vi "DAQ Stop.vi"(8 "Error In":errorcluster caption="错误输入", 10 "Sample Settings":T1={"设备信息"={"初始索引子集"=[], "模拟信号采集通道"="Dev1", "光控设备"="", "数字-光控"="", "数字-供电"="", "光电设备分离？"=FALSE, "光谱保存路径"=path "", "7环?"=FALSE}, "测量控制"={"测头拿起"=FALSE, "是否保存"=FALSE, "测头供电"=TRUE, "测头出光"=TRUE}, "测量"={"每波长测量次数"=5, "波长"=[1050, 1213, 1314, 1409, 1550, 1609], "起始周期"=0, "起始测量周期"=0}, "等待"={"等待时间(s)"=0.0, "等待方式"=FALSE, "每x周期/点等待"=8, "等待时"=enum."无电无光"}, "校准"={"暗电流校准值初值"=[], "温度校准值"=[0.0, 0.0, 0.0, 0.0, 0.0, 0.0, 0.00013, 0.00013, 0.00013, 0.00013, 0.00013, 0.00013]}, "图表相关"={"文件-时间"=""}}) -> (0 "Error Out":errorcluster caption="错误输出")   [LabVIEW 2017, in "UI-无创.lvlib" / "Acquisition.lvlib"]
uses:
  Acquisition.lvlib
  Supports/Sample Settings.ctl
  <vilib>/DAQmx/write.llb/DAQmx Write (Digital U32 1Chan 1Samp).vi
  <vilib>/DAQmx/miscellaneous.llb/DAQmx Fill In Error Info.vi
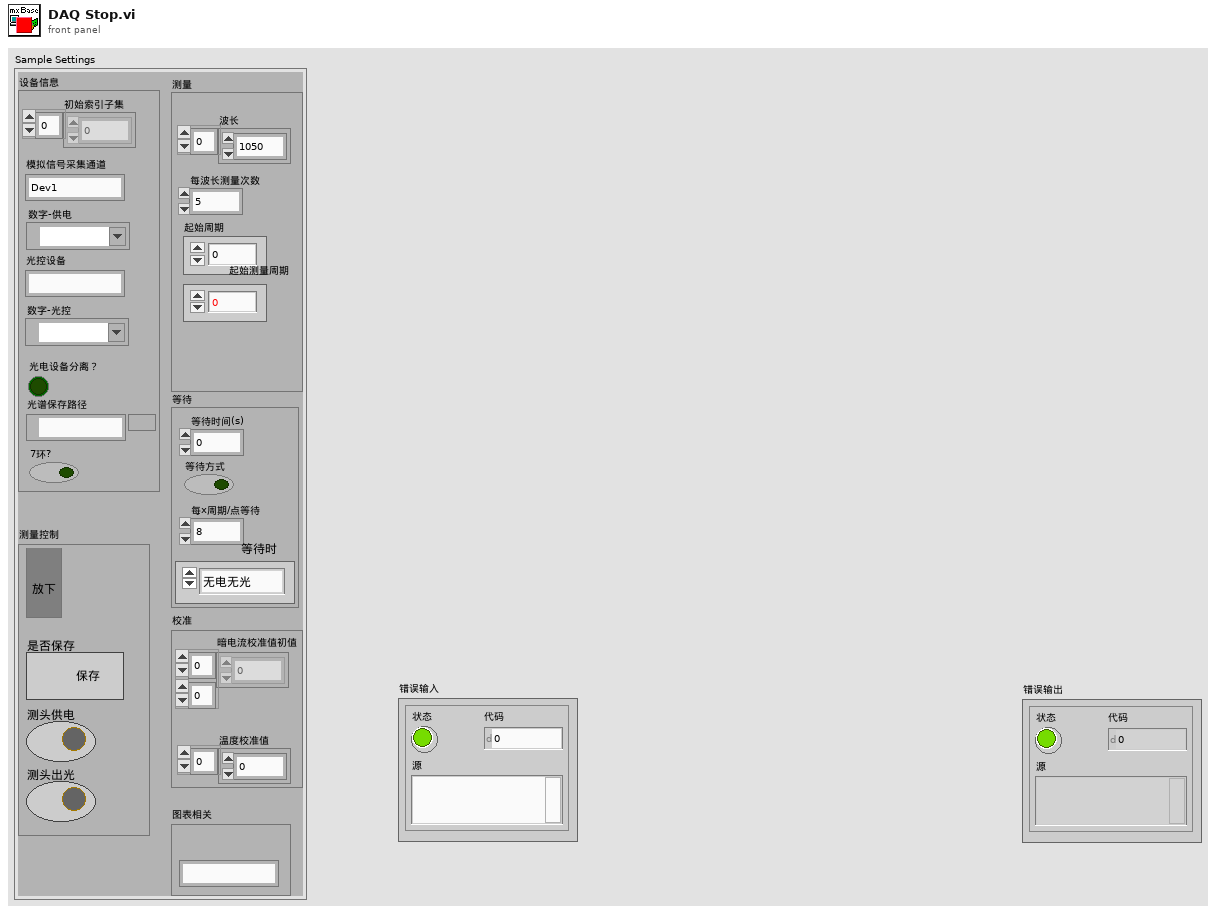
[diagram p1: front panel]
types:
  T1 = typedef "UI-无创.lvlib/Sample Settings.ctl" = cluster{"设备信息":cluster{"初始索引子集":i32[], "模拟信号采集通道":string, "光控设备":string, "数字-光控":refnum<k21>, "数字-供电":refnum<k21>, "光电设备分离？":bool, "光谱保存路径":path, "7环?":bool}, "测量控制":cluster{"测头拿起":bool, "是否保存":bool, "测头供电":bool, "测头出光":bool}, "测量":cluster{"每波长测量次数":i32, "波长":i32[], "起始周期":i32, "起始测量周期":i32}, "等待":cluster{"等待时间(s)":dbl, "等待方式":bool, "每x周期/点等待":i32, "等待时":enum16{"无电无光", "有电无光", "无电有光", "有电有光"}}, "校准":cluster{"暗电流校准值初值":dbl[][], "温度校准值":dbl[]}, "图表相关":cluster{"文件-时间":string}}
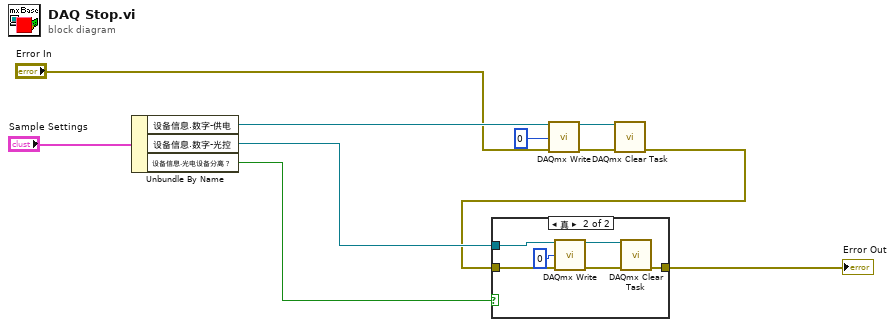
[diagram p0: block diagram]
diagram:
  n1 = Unbundle By Name("Sample Settings") -> ("设备信息.数字-供电"=w7:refnum<k21>, "设备信息.数字-光控"=w5:refnum<k21>, "设备信息.光电设备分离？"=w6:bool)
  n2 = call-poly <vilib>:"DAQmx Write.vi"("task/channels in"=w7, "data"=u32 0, "error in"="Error In") -> ("task out"=w10:refnum<k21>, "error out"=w9:errorcluster)  [unwired: 10 in, 1 out]
  n3 = call <vilib>:"DAQmx Clear Task.vi"("task in"=w10, "error in"=w9) -> ("error out"=w3:errorcluster)  [unwired: 13 in]
  n4 = case shown="真" w6 {
    tunnel: w5 -> [_ w14]
    tunnel: w3 -> [w11 w13]
    tunnel: [w11 w12] -> w1
    frame False {
    }
    frame True {
      n5 = call-poly <vilib>:"DAQmx Write.vi"("task/channels in"=w14, "data"=u32 0, "error in"=w13) -> ("task out"=w15:refnum<k21>, "error out"=w16:errorcluster)  [unwired: 10 in, 1 out]
      n6 = call <vilib>:"DAQmx Clear Task.vi"("task in"=w15, "error in"=w16) -> ("error out"=w12:errorcluster)  [unwired: 13 in]
    }
  }
  "Error Out" <- w1
